vi "Func - Get declared arguments.vi"(6 "arg descriptors":T1(array[cluster]), 7 "InstanceRef":T2, 8 "error in":bool, 9 "max arg num":i32=100, 10 "min arg num":i32=1, 11 "arg list":T3[](array[typedef])) -> (0 "error out":bool, 1 "type list":u32[](array[numeric]), 2 "str list":string[](array[string]), 3 "num list":dbl[](array[numeric]) format="%.3f")   [LabVIEW 2021]
doc: "This VI returns the values of function arguments. It verifies the number of actual arguments and their data types according to provided declaration. Refer to the VI help for more details.\n\n<b>arg list</b> specifies the list of function arguments passed to a FuncVI. Wire it to the same terminal on the FuncVI block diagram.\n\n<b>min arg num</b> and <b>max arg num</b> specify the minimum and the maximum number of arguments allowed.\n\n<B>arg descriptors</B> specifies expected argument types and default values of optional arguments.\n\nFor more information, see help for this VI.\n\n::: CalcExpress Toolkit :::\nCopyright (c) 2000-2026 Konstantin Shifershteyn. All rights reserved."
uses:
  cetypes.llb/CalcExpress Function Argument Info.ctl
  cetypes.llb/CalcExpress Instance RefNum.ctl
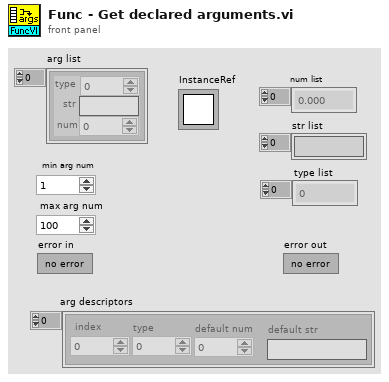
[diagram p1: front panel]
types:
  T1 = cluster{"index":i32, "type":i32, "default num":dbl, "default str":string}[]
  T2 = typedef "CalcExpress Instance RefNum.ctl" = refnum<k1>
  T3 = typedef "CalcExpress Function Argument Info.ctl" = cluster{"type":u32, "str":string, "num":dbl}
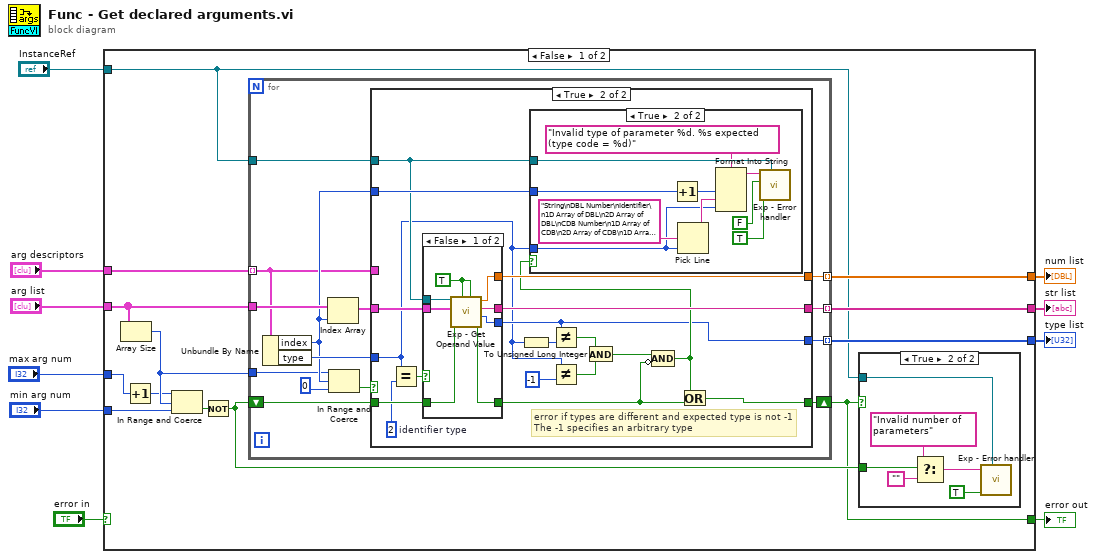
[diagram p0: block diagram]
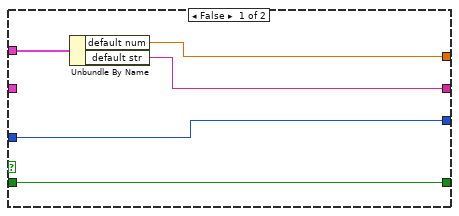
[diagram p3: hidden frame]
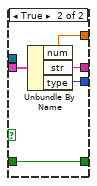
[diagram p5: hidden frame]
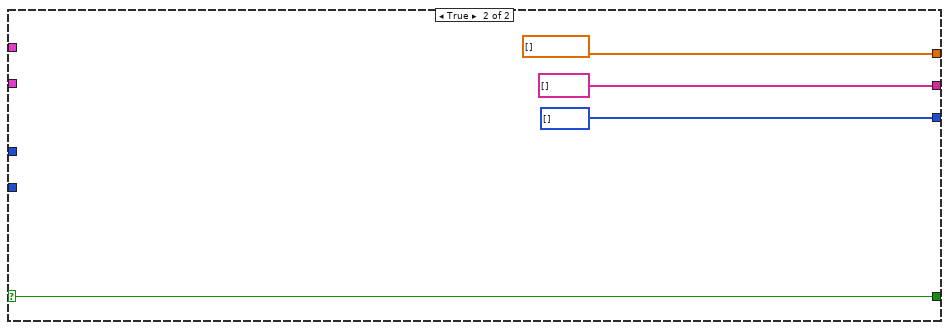
[diagram p6: hidden frame]
diagram:
  n1 = case shown="False" "error in" {
    selector: "error in" -> [_ w90]
    tunnel: [w19 w90] -> w10
    tunnel: [w18 u32[] [] ("type list")] -> w9
    tunnel: [w17 string[] [] ("str list")] -> w8
    tunnel: [w16 dbl[] [] ("num list")] -> w7
    tunnel: "InstanceRef" -> [w15 _]
    tunnel: "arg descriptors" -> [w14 _]
    tunnel: "arg list" -> [w13 _]
    tunnel: "max arg num" -> [w12 _]
    tunnel: "min arg num" -> [w11 _]
    frame False {
      n2 = Array Size(array=w13) -> (size(s)=w23:i32)
      n3 = Increment(x=w12) -> (x+1=w21:i32)
      n4 = In Range and Coerce(upper limit=w21, x=w23, lower limit=w11) -> (In Range?=w20:bool)  [unwired: 1 out]
      n5 = Not(x=w20) -> (.not. x?=w22:bool)
      n6 = for {
        shift-right: [w40] -> w19
        shift-left: w22 -> [w36]
        tunnel: w14 -> [w31] mode=indexing
        tunnel: w13 -> [w43]
        tunnel: w15 -> [w41]
        tunnel: [w39] -> w17 mode=indexing
        tunnel: [w38] -> w16 mode=indexing
        tunnel: w23 -> [w34]
        tunnel: [w30] -> w18 mode=indexing
        n7 = Unbundle By Name(w31) -> ("index"=w35:i32, "type"=w37:i32)
        n8 = Index Array(array=w43, index=w35) -> (element=w42:T3)
        n9 = In Range and Coerce(upper limit=w34, x=w35, lower limit=0 ("lo")) -> (In Range?=w32:bool)  [unwired: 1 out]
        n10 = case shown="True" w32 {
          tunnel: w35 -> [_ w59]
          tunnel: w36 -> [w48 w66]
          tunnel: w37 -> [w44 w49]
          tunnel: [w47 w65] -> w38
          tunnel: [w45 w64] -> w39
          tunnel: [w48 w58] -> w40
          tunnel: w41 -> [_ w57]
          tunnel: w42 -> [_ w63]
          tunnel: w31 -> [w46 _]
          tunnel: [w44 w56] -> w30
          frame False {
            n11 = Unbundle By Name(w46) -> ("default num"=w47:dbl, "default str"=w45:string)
          }
          frame True {
            w51 = 2  # identifier type
            # "error if types are different and expected type is not -1\nThe -1 specifies an arbitrary type"
            n12 = Equal?(x=w49, y=w51) -> (x = y?=w62:bool)
            n13 = case shown="False" w62 {
              tunnel: w66 -> [w82 w86]
              tunnel: w63 -> [w84 w89]
              tunnel: w57 -> [w83 _]
              tunnel: [w78 w86] -> w61
              tunnel: [w81 w88] -> w64
              tunnel: [w80 w87] -> w65
              tunnel: [w77 w85] -> w56
              frame False {
                w79 = TRUE ("may be string ? (F)")
                n14 = call "Exp - Get Operand Value.vi"("ena complex? (F)"=w79, "ena string? (F)"=w79, "error in"=w82, "op info"=w84, "InstanceRef"=w83) -> ("error out"=w78:bool, "type"=w77:u32, "str"=w81:string, "num"=w80:dbl)  [unwired: 1 in]
              }
              frame True {
                n15 = Unbundle By Name(w89) -> ("num"=w87:dbl, "str"=w88:string, "type"=w85:u32)
              }
            }
            n16 = To Unsigned Long Integer(number=w49) -> (unsigned 32bit integer=w50:u32)
            n17 = Not Equal?(x=w56, y=w50) -> (x != y?=w55:bool)
            n18 = Not Equal?(x=w49, y=-1) -> (x != y?=w52:bool)
            n19 = And(x=w55, y=w52) -> (x .and. y?=w54:bool)
            n20 = Compound Arithmetic op=AND(w54, invert w61) -> (w60:bool)
            n21 = case shown="True" w60 {
              tunnel: w59 -> [_ w73]
              tunnel: w49 -> [_ w67]
              tunnel: w57 -> [_ w72]
              frame False {
              }
              frame True {
                n22 = Increment(x=w73) -> (x+1=w75:i32)
                n23 = Pick Line(multi-line string="String\nDBL Number\nIdentifier\n1D Array of DBL\n2D Array of DBL\nCDB Number\n1D Array of CDB\n2D Array of CDB\n1D Array of String\n2D Array of String\n", line index=w67) -> (output string=w70:string)  [unwired: 1 in]
                n24 = Format Into String(format string="Invalid type of parameter %d. %s expected (type code = %d)", w75, w70, w67) -> (resulting string=w76:string)  [unwired: 2 in, 1 out]
                n25 = call "Exp - Error handler.vi"("InstanceRef"=w72, "error in"=TRUE, "add FuncName (T)"=FALSE, "error message in"=w76) -> ()  [unwired: 5 in, 3 out]
              }
            }
            n26 = Or(x=w60, y=w61) -> (x .or. y?=w58:bool)
          }
        }
      }
      n27 = case shown="True" w19 {
        tunnel: w22 -> [_ w29]
        tunnel: w15 -> [_ w24]
        frame False {
        }
        frame True {
          n28 = Select(t="Invalid number of parameters" ("ErrStr"), s=w29, f="" ("Empty String Constant")) -> (s? t:f=w25:string)
          n29 = call "Exp - Error handler.vi"("InstanceRef"=w24, "error in"=TRUE, "error message in"=w25) -> ()  [unwired: 6 in, 3 out]
        }
      }
    }
    frame True {
    }
  }
  "error out" <- w10
  "num list" <- w7
  "str list" <- w8
  "type list" <- w9
